vi "Test_Displays_Direct.vi"(8 "error in":errorcluster) -> (0 "error out":errorcluster)   [LabVIEW 2026]
doc: "No-AF probe: configures the executor object with refs to this VI's own Status and Step Index indicators, writes Status via Write Status, calls Update Displays, and reads nothing back - the indicators must show the written values after the run."
uses:
  src/Executor/Sequence Executor.lvclass
  src/Executor/Sequence Executor.lvclass/Sequence Executor.ctl
panel:
  out "Step Index":i32
  out "Status":string
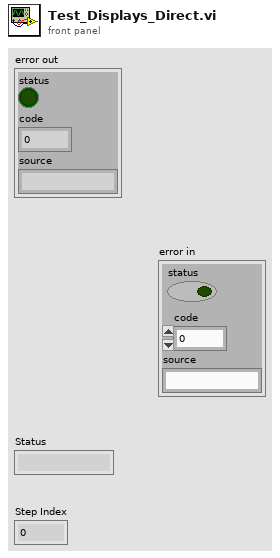
[diagram p1: front panel]
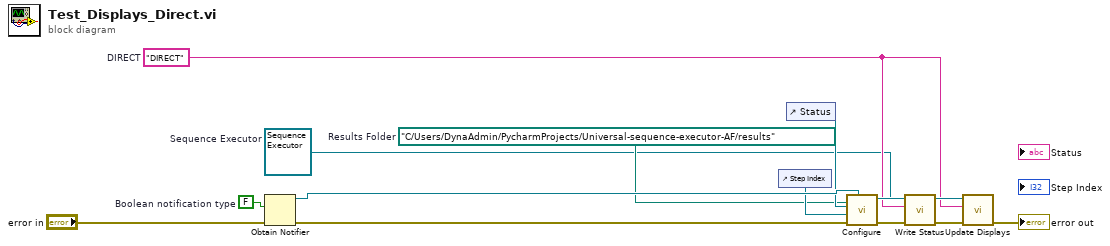
[diagram p0: block diagram]
diagram:
  w4 = path "C:/Users/DynaAdmin/PycharmProjects/Universal-sequence-executor-AF/results"  # Results Folder
  w3 = "DIRECT"  # DIRECT
  w2 = FALSE  # Boolean notification type
  w1 = refnum<class "Sequence Executor.lvclass"> refnum  # Sequence Executor
  n1 = Obtain Notifier(notification data type=w2, error in (no error)="error in") -> (notifier out=w8:refnum<notifier>, error out=w9:errorcluster)  [unwired: 2 in, 1 out]
  n2 = control-ref of="Step Index"() -> (w7:refnum<vi>)
  n3 = control-ref of="Status"() -> (w6:refnum<vi>)
  n4 = call "Configure.vi"("Results Folder"=w4, "Stopped Notification"=w8, "error in"=w9, "Step Index Display"=w7, "Status Display"=w6, "Sequence Executor in"=w1) -> ("error out"=w11:errorcluster, "Sequence Executor out"=w10:refnum<class "Sequence Executor.lvclass">)  [unwired: 4 in]
  n5 = call "Write Status.vi"("error in (no error)"=w11, "Status"=w3, "Sequence Executor in"=w10) -> ("error out"=w13:errorcluster, "Sequence Executor out"=w12:refnum<class "Sequence Executor.lvclass">)  [unwired: 7 in]
  n6 = call "Update Displays.vi"("error in"=w13, "Status"=w3, "Sequence Executor in"=w12) -> ("error out"=→"error out":errorcluster)  [unwired: 7 in, 1 out]
